vi "Route.vi"(8 "error in (no error)":errorcluster caption="에러 입력(에러 없음)", 11 "Instrument Manager 입력":refnum<class "Instrument Manager.lvclass">) -> (0 "error out":errorcluster caption="에러 출력", 3 "Instrument Manager 출력":refnum<class "Instrument Manager.lvclass">)   [LabVIEW 2023, in "Instrument Manager.lvclass"]
uses:
  Instrument Manager.lvclass
  Instrument Manager.lvclass/Instrument Manager.ctl
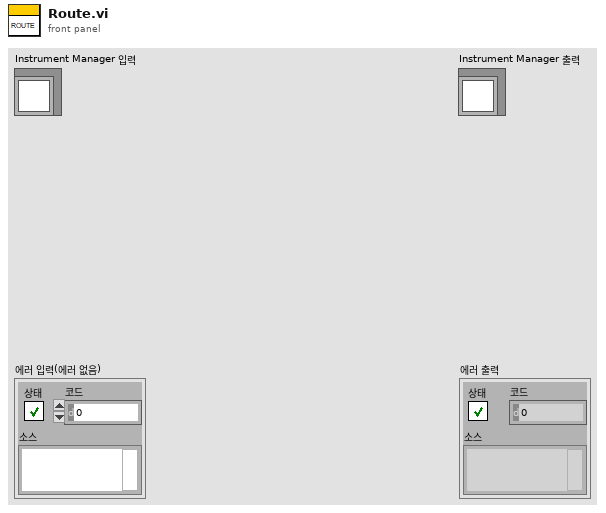
[diagram p1: front panel]
types:
  T1 = cluster{"Reader Q":refnum<queue>, "Writer Q":refnum<queue>}
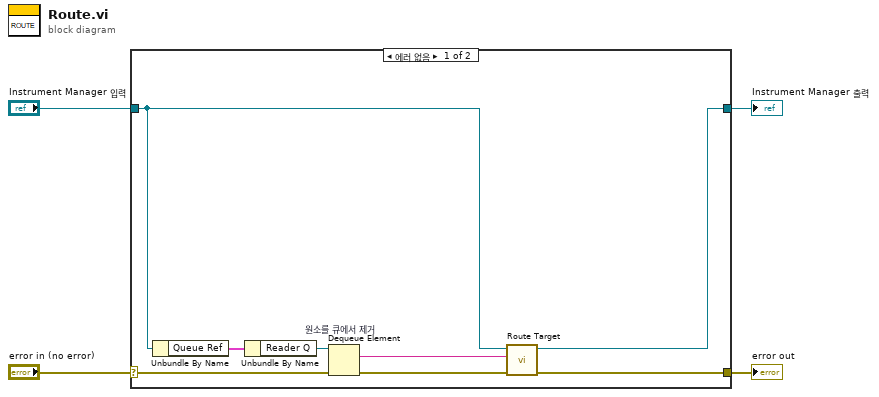
[diagram p0: block diagram]
diagram:
  n1 = case shown="에러 없음" "error in (no error)" {
    selector: "error in (no error)" -> [w10 w14]
    tunnel: [w8 w14] -> w3
    tunnel: [w5 w13] -> w1
    tunnel: "Instrument Manager 입력" -> [w6 w13]
    frame No Error {
      n2 = Unbundle By Name(w6) -> ("Queue Ref"=w12:T1)
      n3 = Unbundle By Name(w12) -> ("Reader Q"=w11:refnum<queue>)
      n4 = Dequeue Element "원소를 큐에서 제거"(queue=w11, error in (no error)=w10) -> (element=w7:string, error out=w9:errorcluster)  [unwired: 1 in, 2 out]
      n5 = call "Route Target.vi"("error in (no error)"=w9, "Request"=w7, "Instrument Manager 입력"=w6) -> ("error out"=w8:errorcluster, "Instrument Manager 출력"=w5:refnum<class "Instrument Manager.lvclass">)  [unwired: 7 in]
    }
    frame Error {
    }
  }
  "error out" <- w3
  "Instrument Manager 출력" <- w1
